vi "Runners_Data.vi"(8 "error in":errorcluster) -> (0 "error out":errorcluster, 3 "Runners Data Out":T1)   [LabVIEW 2025]
uses:
  Controls/Runners_Data.ctl
panel:
  in  "OK Button":bool
  in  "Runners Data":T1
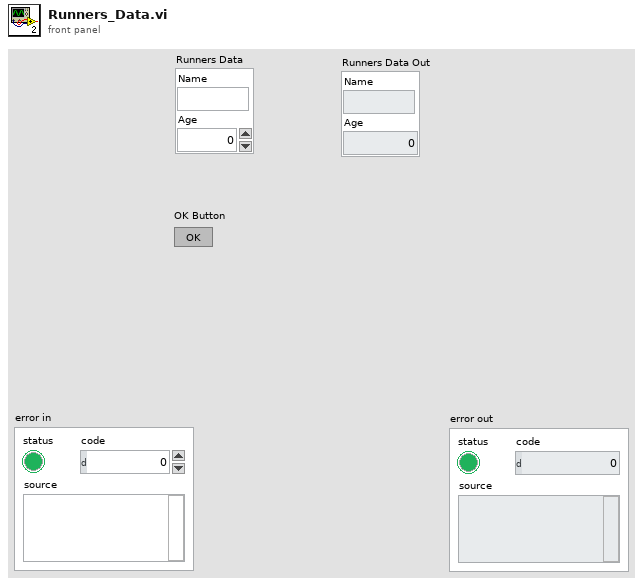
[diagram p1: front panel]
types:
  T1 = typedef "Runners_Data.ctl" = cluster{"Name":string, "Age":i32}
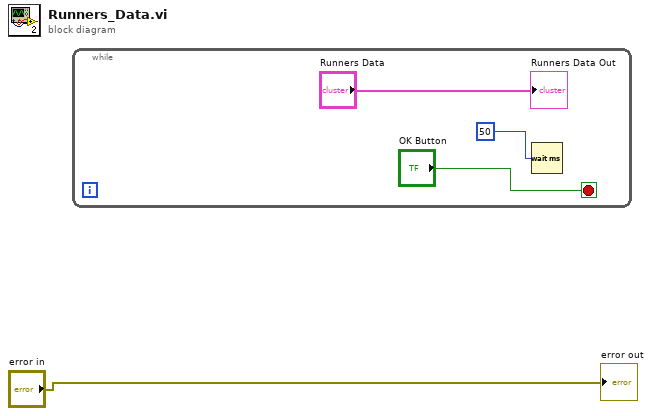
[diagram p0: block diagram]
diagram:
  n1 = while {
    stop <- "OK Button" stop-if-true
    n2 = Wait (ms)(milliseconds to wait=u32 50) -> ()  [unwired: 1 out]
    "Runners Data Out" <- "Runners Data"
  }
  "error out" <- "error in"
